vi "Build Preview.vi"(0 "# Of Loops":u32, 5 "Program":T1(array[cluster]), 7 "Loop ?":cluster{i32, i32}, 9 "Initial Value":dbl, 11 "error in (no error)":errorcluster, 12 "Average During Loop ?":bool) -> (1 "Stage Values":i32[](array[numeric]), 3 "Plots Out":cluster{dbl[], dbl[]}[](array[cluster]), 4 "Storage Locations Out":i32[](array[numeric]), 6 "Y Values Out":dbl[](array[numeric]), 10 "Measure ? Out":bool[](array[boolean]), 14 "Direction Out":bool[](array[boolean]), 15 "error out":errorcluster)   [LabVIEW 2012, in "Multi Segment Waveform.xctl"]
doc: "Builds a set of X-Y plots based on the current program and loop settings ."
uses:
  Multi Segment Waveform.xctl
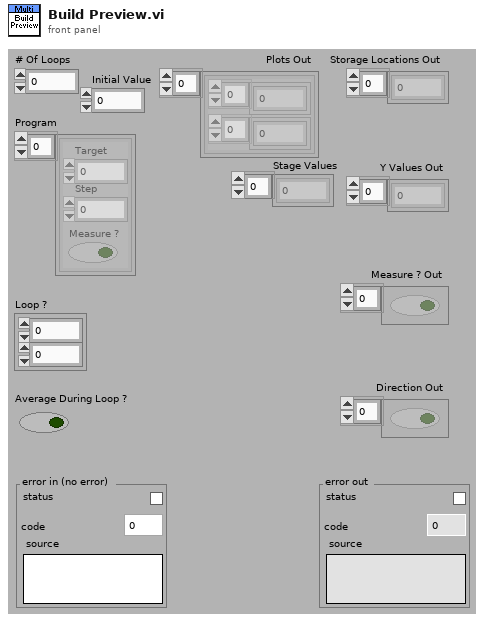
[diagram p1: front panel]
types:
  T1 = cluster{"Target":dbl, "Step":dbl, "Measure ?":bool}[]
  T2 = cluster{"Storage Locs":i32[], "Measure":bool[], "Field":dbl[], "Direction":bool[]}
  T3 = cluster{"Target":dbl, "Step":dbl, "Measure ?":bool}
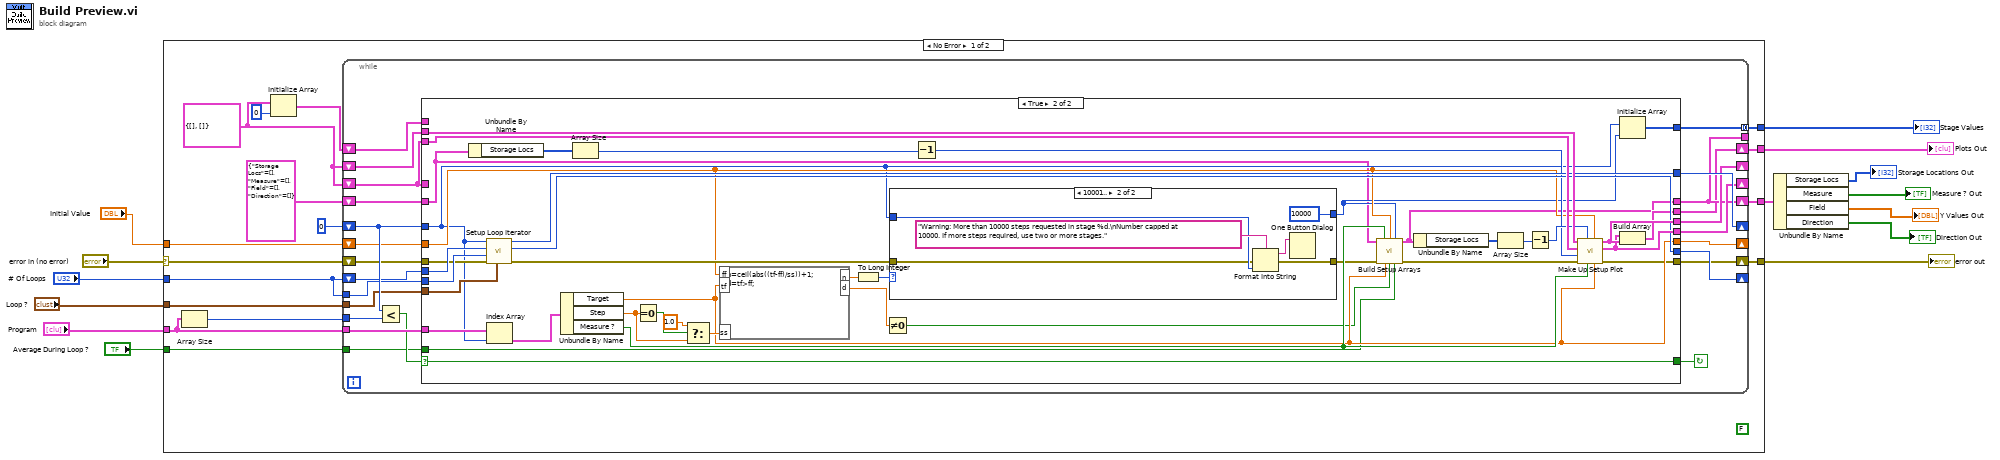
[diagram p0: block diagram]
diagram:
  n1 = case shown="No Error" "error in (no error)" {
    selector: "error in (no error)" -> [w19 w113]
    tunnel: [w27 _] -> w14
    tunnel: "Average During Loop ?" -> [w26 _]
    tunnel: "Loop ?" -> [w25 _]
    tunnel: "Program" -> [w24 _]
    tunnel: "# Of Loops" -> [w21 _]
    tunnel: [w20 _] -> w6
    tunnel: [w18 w113] -> w8
    tunnel: [w17 _] -> w7
    tunnel: "Initial Value" -> [w15 _]
    frame No Error {
      w28 = cluster{dbl[], dbl[]} {[], []}
      (unwired) FALSE
      n2 = Array Size(array=w24) -> (size(s)=w22:i32)
      n3 = Initialize Array(w28, 0 ("dimension size")) -> (w29:cluster{dbl[], dbl[]}[])
      n4 = while {
        tunnel: [w38] -> _
        shift-left: T2 {"Storage Locs"=[], "Measure"=[], "Field"=[], "Direction"=[]} ("Preview Out") -> [w39]
        shift-right: [w38] -> w20
        tunnel: w21 -> [w40]
        shift-left: w28 -> [w44]
        shift-right: [w43] -> _
        shift-left: w28 -> [w41]
        shift-right: [w42] -> _
        shift-left: w21 -> [w49]
        shift-right: [w48] -> _
        tunnel: w22 -> [w52]
        shift-left: 0 -> [w54]
        shift-right: [w47] -> _
        shift-left: w15 -> [w46]
        shift-right: [w45] -> _
        tunnel: w24 -> [w53]
        tunnel: w25 -> [w37]
        tunnel: w26 -> [w35]
        shift-right: [w36] -> w27
        shift-left: w29 -> [w34]
        shift-right: [w33] -> w18
        shift-left: w19 -> [w32]
        tunnel: [w31] -> w17 mode=concatenating
        stop <- w50 continue-if-true
        n5 = Less?(x=w54, y=w52) -> (x < y?=w51:bool)
        n6 = case shown="True" w51 {
          selector: w51 -> [w63 w94]
          tunnel: w54 -> [w61 w69]
          tunnel: w53 -> [_ w104]
          tunnel: [w63 w94] -> w50
          tunnel: w49 -> [w62 w97]
          tunnel: [w62 w96] -> w48
          tunnel: [w61 w95] -> w47
          tunnel: w46 -> [w60 w75]
          tunnel: [w60 w80] -> w45
          tunnel: w41 -> [_ w100]
          tunnel: w44 -> [w58 w99]
          tunnel: [w58 w102] -> w43
          tunnel: [w59 w101] -> w42
          tunnel: w41 -> [w59 _]
          tunnel: w40 -> [_ w98]
          tunnel: w39 -> [w57 w67]
          tunnel: [w57 w65] -> w38
          tunnel: w37 -> [_ w79]
          tunnel: [w56 w86] -> w36
          tunnel: w35 -> [_ w73]
          tunnel: w34 -> [w56 _]
          tunnel: [w55 w71] -> w33
          tunnel: w32 -> [w55 w78]
          tunnel: [_ w68] -> w31
          frame False {
          }
          frame True {
            n7 = Unbundle By Name(w67) -> ("Storage Locs"=w66:i32[])
            n8 = call "Setup Loop Iterator.vi"("Loop"=w79, "error in (no error)"=w78, "Total Loops"=w98, "Loop Iterator"=w97, "Previous Line"=w69) -> ("error out"=w77:errorcluster, "Loop Iterator Out"=w96:u32, "Line Iterator Out"=w95:i32)  [unwired: 4 out]
            n9 = Index Array(array=w104, index=w69) -> (element=w103:T3)
            n10 = Unbundle By Name(w103) -> ("Target"=w80:dbl, "Step"=w83:dbl, "Measure ?"=w87:bool)
            n11 = Array Size(array=w66) -> (size(s)=w89:i32)
            n12 = Equal To 0?(x=w83) -> (x = 0?=w85:bool)
            n13 = Select(t=1.0, s=w85, f=w83) -> (s? t:f=w82:dbl)
            n14 = formula code="n=ceil(abs((tf-ff)/ss))+1;\nd=tf>ff;"("ff"=w75, "tf"=w80, "ss"=w82) -> ("n"=w92:dbl, "d"=w93:dbl)
            n15 = To Long Integer(number=w92) -> (32bit integer=w81:i32)
            n16 = Not Equal To 0?(x=w93) -> (x != 0?=w74:bool)
            n17 = case shown="10001.." w81 {
              selector: w81 -> [w106 _]
              tunnel: [w106 10000] -> w70
              tunnel: w69 -> [_ w110]
              tunnel: w77 -> [w105 w108]
              tunnel: [w105 w107] -> w76
              frame ..10000 {
              }
              frame 10001.. {
                n18 = Format Into String(format string="Warning: More than 10000 steps requested in stage %d.\nNumber capped at 10000. If more steps required, use two or more stages.", error in=w108, w110) -> (resulting string=w109:string, error out=w107:errorcluster)  [unwired: 1 in]
                n19 = One Button Dialog(message=w109) -> ()  [unwired: 2 out]
              }
            }
            n20 = Decrement(x=w89) -> (x-1=w88:i32)
            n21 = call "Build Setup Arrays.vi"("Preview In"=w67, "Measure ?"=w87, "First Field"=w75, "N Points"=w70, "error in (no error)"=w76, "Last Field"=w80, "Direction"=w74, "Average During Loop ?"=w73) -> ("Preview Out"=w65:T2, "error out"=w72:errorcluster)  [unwired: 3 in, 3 out]
            n22 = Unbundle By Name(w65) -> ("Storage Locs"=w64:i32[])
            n23 = Array Size(array=w64) -> (size(s)=w91:i32)
            n24 = Decrement(x=w91) -> (x-1=w90:i32)
            n25 = call "Make Up Setup Plot.vi"("End Field"=w80, "Start Field"=w75, "Put in plot 1"=w87, "End X"=w90, "error in (no error)"=w72, "Start X"=w88, "Plot 1 In"=w100, "Plot 2 In"=w99) -> ("error out"=w71:errorcluster, "Plot 1 Out"=w101:cluster{dbl[], dbl[]}, "Plot 2 Out"=w102:cluster{dbl[], dbl[]})  [unwired: 1 out]
            n26 = Initialize Array(w69, w70) -> (w68:i32[])
            n27 = Build Array(w101, w102) -> (w86:cluster{dbl[], dbl[]}[])
          }
        }
      }
    }
    frame Error {
    }
  }
  "Plots Out" <- w14
  "error out" <- w8
  "Stage Values" <- w7
  n28 = Unbundle By Name(w6) -> ("Storage Locs"=→"Storage Locations Out":i32[], "Measure"=→"Measure ? Out":bool[], "Field"=→"Y Values Out":dbl[], "Direction"=→"Direction Out":bool[])
